vi "Element Init.vi"(7 "VolatusAPI":refnum<class "VolatusAPI.lvclass">, 8 "error in (no error)":errorcluster, 10 "JSON":string, 11 "GaugeIndicator in":refnum<class "GaugeIndicator.lvclass">) -> (0 "error out":errorcluster, 3 "GaugeIndicator out":refnum<class "GaugeIndicator.lvclass">)   [LabVIEW 2020, in "VolatusGUIElements.lvlib" / "GaugeIndicator.lvclass"]
uses:
  GaugeIndicator.lvclass
  Volatus/VolatusAPI/VolatusAPI.lvclass
  GaugeIndicator.lvclass/GaugeIndicator.ctl
  lv-cdm/CDM-Config/Config-JSON/Config-JSON.lvclass
  lv-cdm/CDM-Config/Config Manager/Config Manager.lvclass
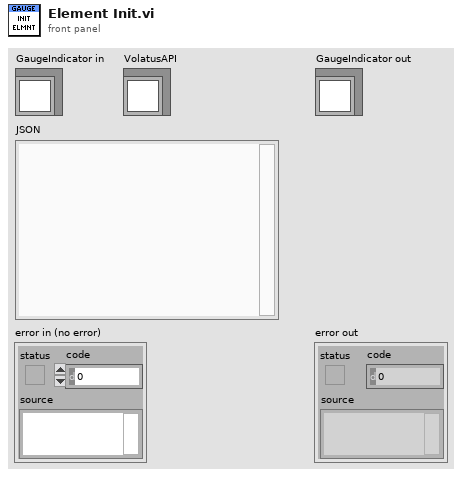
[diagram p1: front panel]
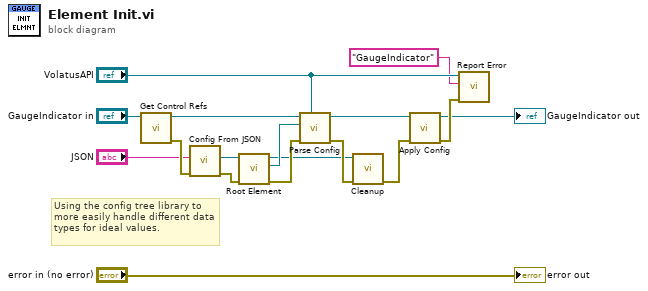
[diagram p0: block diagram]
diagram:
  # "Using the config tree library to more easily handle different data types for ideal values."
  n1 = call "Get Control Refs.vi"("GaugeIndicator in"="GaugeIndicator in") -> ("error out"=w15:errorcluster, "GaugeIndicator out"=w12:refnum<class "GaugeIndicator.lvclass">)  [unwired: 9 in]
  n2 = call "Config From JSON.vi"("error in (no error)"=w15, "JSON"="JSON") -> ("error out"=w9:errorcluster, "Config"=w10:refnum<class "Config Manager.lvclass">)  [unwired: 8 in]
  n3 = call "Root Element.vi"("error in (no error)"=w9, "Config Manager in"=w10) -> ("error out"=w6:errorcluster, "Root Element"=w7:refnum<class "Config Element.lvclass">, "Config Manager out"=w5:refnum<class "Config Manager.lvclass">)  [unwired: 7 in]
  n4 = call "Parse Config.vi"("VolatusAPI"="VolatusAPI", "error in (no error)"=w6, "Config Element"=w7, "GaugeIndicator in"=w12) -> ("error out"=w16:errorcluster, "GaugeIndicator out"=w8:refnum<class "GaugeIndicator.lvclass">)  [unwired: 6 in]
  n5 = call "Cleanup.vi"("error in (no error)"=w16, "Config Manager in"=w5) -> ("error out"=w3:errorcluster)  [unwired: 9 in]
  n6 = call "Apply Config.vi"("error in (no error)"=w3, "GaugeIndicator in"=w8) -> ("error out"=w17:errorcluster, "GaugeIndicator out"=→"GaugeIndicator out":refnum<class "GaugeIndicator.lvclass">)  [unwired: 8 in]
  n7 = call "Report Error.vi"("error in (no error)"=w17, "Context"="GaugeIndicator", "VolatusAPI in"="VolatusAPI") -> ()  [unwired: 7 in, 2 out]
  "error out" <- "error in (no error)"
